vi "MoveMouseCursorOnCtrl.vi"(0 "VI Reference In":refnum<vi>, 5 "Control Ref In":refnum<vi>, 7 "Offset":i32, 11 "Error In":errorcluster) -> (4 "VI Reference Out":refnum<vi>, 6 "Control Ref Out":refnum<vi>, 15 "Error Out":errorcluster)   [LabVIEW 2019, in "Drona.lvlib"]
doc: "This VI moves mouse cursor position to the given control references position"
uses:
  Drona.lvlib
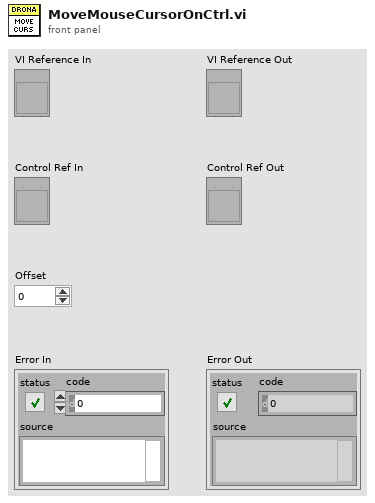
[diagram p1: front panel]
types:
  T1 = typedef "LVRectTypeDef.ctl" = cluster{"Left":i16, "Top":i16, "Right":i16, "Bottom":i16}
  T2 = typedef "LVPositionTypeDef.ctl" = cluster{"Left":i32, "Top":i32}
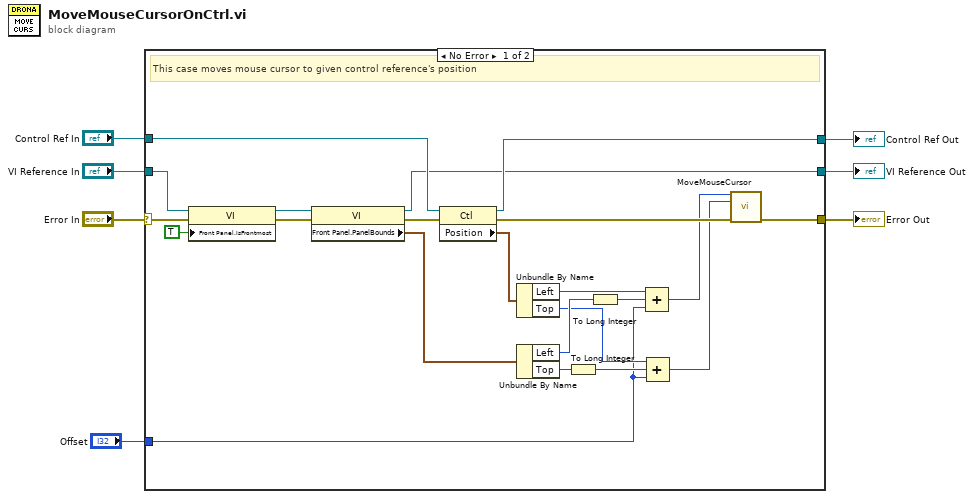
[diagram p0: block diagram]
diagram:
  n1 = case shown="No Error" "Error In" {
    selector: "Error In" -> [w29 w32]
    tunnel: "Control Ref In" -> [w27 w30]
    tunnel: "VI Reference In" -> [w10 w31]
    tunnel: "Offset" -> [w18 _]
    tunnel: [w14 w32] -> w3
    tunnel: [w13 w30] -> w2
    tunnel: [w12 w31] -> w1
    frame No Error {
      # "This case moves mouse cursor to given control reference's position"
      n2 = property class="VI"(reference=w10, error in=w29, "Front Panel.IsFrontmost"=TRUE ("Front Panel Window:Is Frontmost")) -> (reference out=w9:refnum<vi>, error out=w11:errorcluster)
      n3 = property class="VI"(reference=w9, error in=w11) -> (reference out=w12:refnum<vi>, error out=w28:errorcluster, "Front Panel.PanelBounds"=w26:T1)
      n4 = property class="Ctl"(reference=w27, error in=w28) -> (reference out=w13:refnum<vi>, error out=w17:errorcluster, "Position"=w25:T2)
      n5 = Unbundle By Name(w25) -> ("Left"=w24:i32, "Top"=w20:i32)
      n6 = Unbundle By Name(w26) -> ("Left"=w23:i16, "Top"=w21:i16)
      n7 = To Long Integer(number=w21) -> (32bit integer=w19:i32)
      n8 = To Long Integer(number=w23) -> (32bit integer=w22:i32)
      n9 = Compound Arithmetic op=ADD(w24, w22, w18) -> (w16:i32)
      n10 = Compound Arithmetic op=ADD(w20, w19, w18) -> (w15:i32)
      n11 = call "MoveMouseCursor.vi"("Left Position"=w16, "Right Position"=w15, "Error In"=w17) -> ("Error Out"=w14:errorcluster)  [unwired: 12 in]
    }
    frame Error {
      # "If error, this case pass that error message only"
    }
  }
  "Error Out" <- w3
  "Control Ref Out" <- w2
  "VI Reference Out" <- w1
